vi "GetVarFromConnection.vi"   [LabVIEW 2026]
uses:
  <vilib>/vision/Image Controls.llb/IMAQ Image.ctl
  Typedefs/System_State.ctl
  Variables/ComGlobalVars.vi
types:
  T1 = typedef "IMAQ Image.ctl" = refnum<image>
  T2 = typedef "System_State.ctl" = u16
  T3 = cluster{i32, i32, i32, i32, dbl, bool, bool, bool, bool, string, "System State":T2}
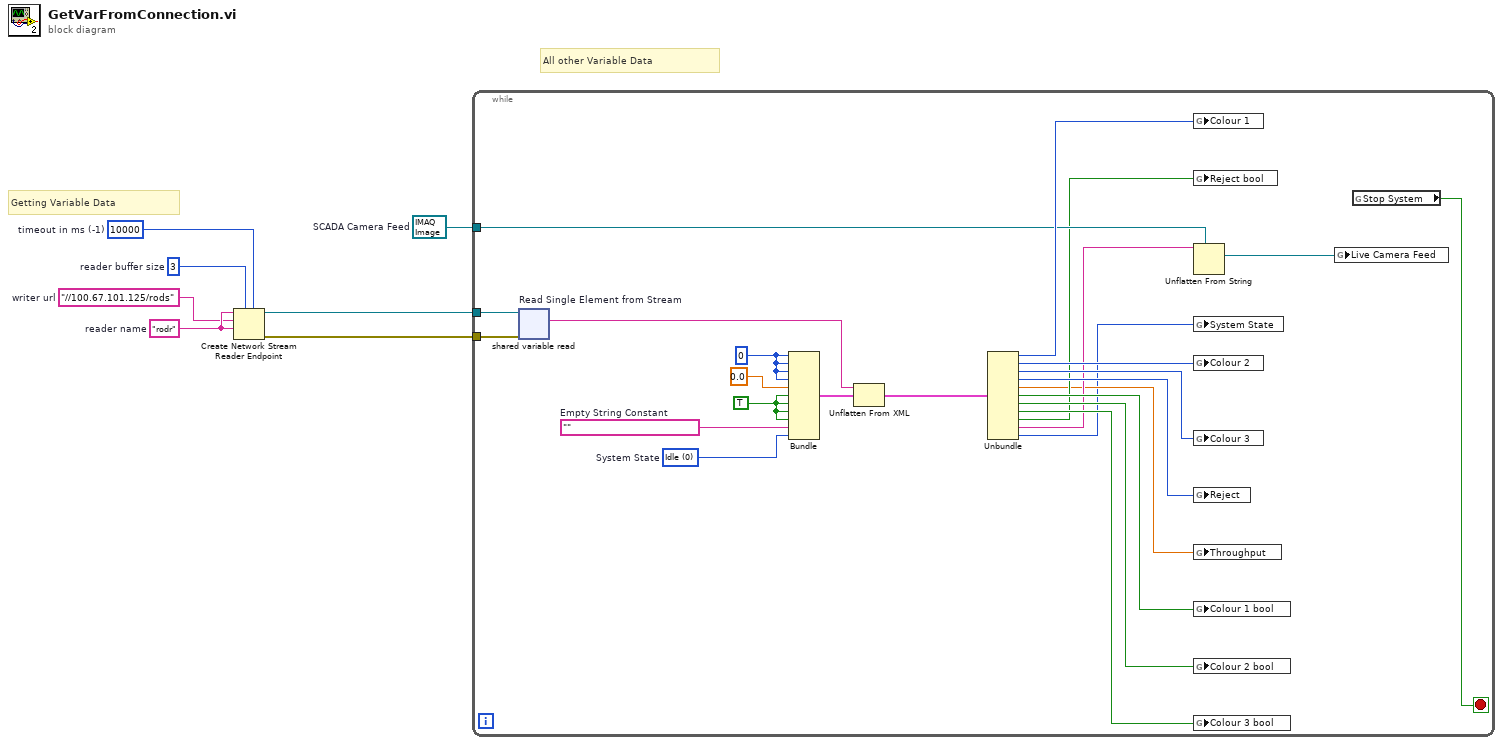
[diagram p0: block diagram]
diagram:
  w4 = 3  # reader buffer size
  w5 = 10000  # timeout in ms (-1)
  w6 = "//100.67.101.125/rods"  # writer url
  w7 = "rodr"  # reader name
  w1 = T1 refnum  # SCADA Camera Feed
  # "Getting Variable Data"
  # "All other Variable Data"
  n1 = Create Network Stream Reader Endpoint(5:w5, 7:w4, 9:w7, 10:w6, 11:w7) -> (0:w2:errorcluster, 3:w3:refnum<k21>)  [unwired: 2 in]
  n2 = while {
    tunnel: w3 -> [w31]
    tunnel: w2 -> [w30]
    tunnel: w1 -> [w20]
    stop <- w9 stop-if-true
    w11 = T2 0 items=["Idle", "Classify", "Sort"]  # System State
    w14 = ""  # Empty String Constant
    w25 = TRUE
    w26 = 0
    n3 = shared-variable-read "Read Single Element from Stream"(w31, w30) -> (w29:string)  [unwired: 1 in, 3 out]
    n4 = Bundle "Bundle"(w26, w26, w26, w26, 0.0, w25, w25, w25, w25, w14, "System State"=w11) -> (w27:T3)  [unwired: 1 in]
    n5 = Unflatten From XML(xml string=w29, type=w27) -> (value=w28:T3)  [unwired: 1 in, 1 out]
    n6 = Unbundle "Unbundle"(w28) -> (w24:i32, w23:i32, w22:i32, w21:i32, w12:dbl, w19:bool, w18:bool, w17:bool, w16:bool, w13:string, "System State"=w10:T2)
    n7 = global write "ComGlobalVars.vi" "Colour 1"(w24) -> ()
    n8 = global write "ComGlobalVars.vi" "Reject bool"(w16) -> ()
    n9 = Unflatten From String(type=w20, binary string=w13) -> (value=w8:T1)  [unwired: 3 in, 2 out]
    n10 = global write "ComGlobalVars.vi" "System State"(w10) -> ()
    n11 = global write "ComGlobalVars.vi" "Colour 2"(w23) -> ()
    n12 = global write "ComGlobalVars.vi" "Colour 3"(w22) -> ()
    n13 = global write "ComGlobalVars.vi" "Reject"(w21) -> ()
    n14 = global write "ComGlobalVars.vi" "Throughput"(w12) -> ()
    n15 = global write "ComGlobalVars.vi" "Colour 1 bool"(w19) -> ()
    n16 = global write "ComGlobalVars.vi" "Colour 2 bool"(w18) -> ()
    n17 = global write "ComGlobalVars.vi" "Colour 3 bool"(w17) -> ()
    n18 = global write "ComGlobalVars.vi" "Live Camera Feed"(w8) -> ()
    n19 = global read "ComGlobalVars.vi" "Stop System"() -> (w9:bool)
  }
